vi "Remove Subscriber.vi"(8 "error in (no error)":errorcluster, 10 "Publisher to Remove":string, 11 "CIF_CIPC_Chn in":refnum<class "CIF_Iceoryx_Chn.lvclass">) -> (0 "error out":errorcluster, 3 "CIF_CIPC_Chn out":refnum<class "CIF_Iceoryx_Chn.lvclass">)   [LabVIEW 2021, in "CIF_Iceoryx_Chn.lvclass"]
uses:
  CIF_Iceoryx_Chn.lvclass
  CIF_Iceoryx_Chn.lvclass/CIF_Iceoryx_Chn.ctl
  CIFChannels/CIFChannels.lvclass
  D:/dev/Packages/CIF_Channels_Core/src/CIFChannels/CIFChannels.lvclass
  D:/dev/Packages/CIF_Channels_Core/src/Iceorxy_Channels/CIF_Iceoryx_Chan/CIF_Iceoryx_Chn.lvclass
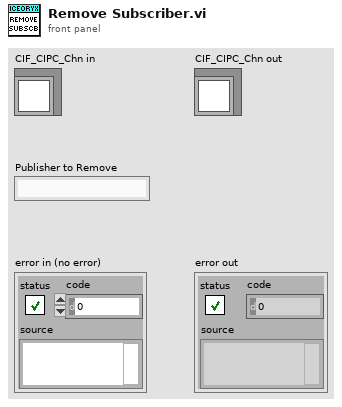
[diagram p1: front panel]
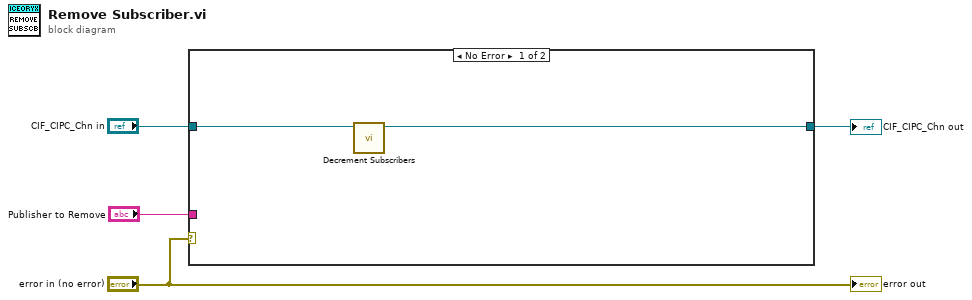
[diagram p0: block diagram]
diagram:
  n1 = case shown="No Error" "error in (no error)" {
    tunnel: "Publisher to Remove" -> [_ _]
    tunnel: "CIF_CIPC_Chn in" -> [w6 w7]
    tunnel: [w5 w7] -> w2
    frame No Error {
      n2 = call "Decrement Subscribers.vi"("CIFChannels in"=w6) -> ("CIFChannels out"=w5:refnum<class "CIF_Iceoryx_Chn.lvclass">)  [unwired: 9 in, 1 out]
    }
    frame Error {
    }
  }
  "CIF_CIPC_Chn out" <- w2
  "error out" <- "error in (no error)"
